vi "Rabi Start.vi"() -> ()   [LabVIEW 2024]
panel:
  in  "Use delay commands?":bool
  in  "T set":string="5E3"
  in  "B Gate Delay":dbl=1.837e-05
  in  "A Gate Delay":dbl=6.308e-06
  in  "stop":bool
  out "At Pass":i32
  in  "MW":dbl=2e-09
  out "Current MW":dbl
  in  "N":dbl=5.0
  out "XY Graph":cluster{"Y":dbl[], "Y":dbl[]}[](graph)
  out "At step":i32
  out "data":dbl[](array[numeric])
  out "A Gate":dbl[][](array[numeric])
  out "B Gate":dbl[][](array[numeric])
  out "DATA":dbl[][](array[numeric])
  in  "Number of steps":i32=500
  in  "Number of individual passes?":i32=10
  in  "Frequency in MHz":string="f2585"
  in  "file path (use dialog)":path=path "C:/Users/Crawford Group/Desktop/DATA (labVIEW Writes)/Rabi/B Gate.txt"
  in  "file path (use dialog) 2":path=path "C:/Users/Crawford Group/Desktop/DATA (labVIEW Writes)/Rabi/A Gate.txt"
  in  "file path (use dialog) 3":path=path "C:/Users/Crawford Group/Desktop/DATA (labVIEW Writes)/Rabi/Averaged.txt"
  # "A gate delay typically at 0.528us\nB gate delay typically at 10.51us"
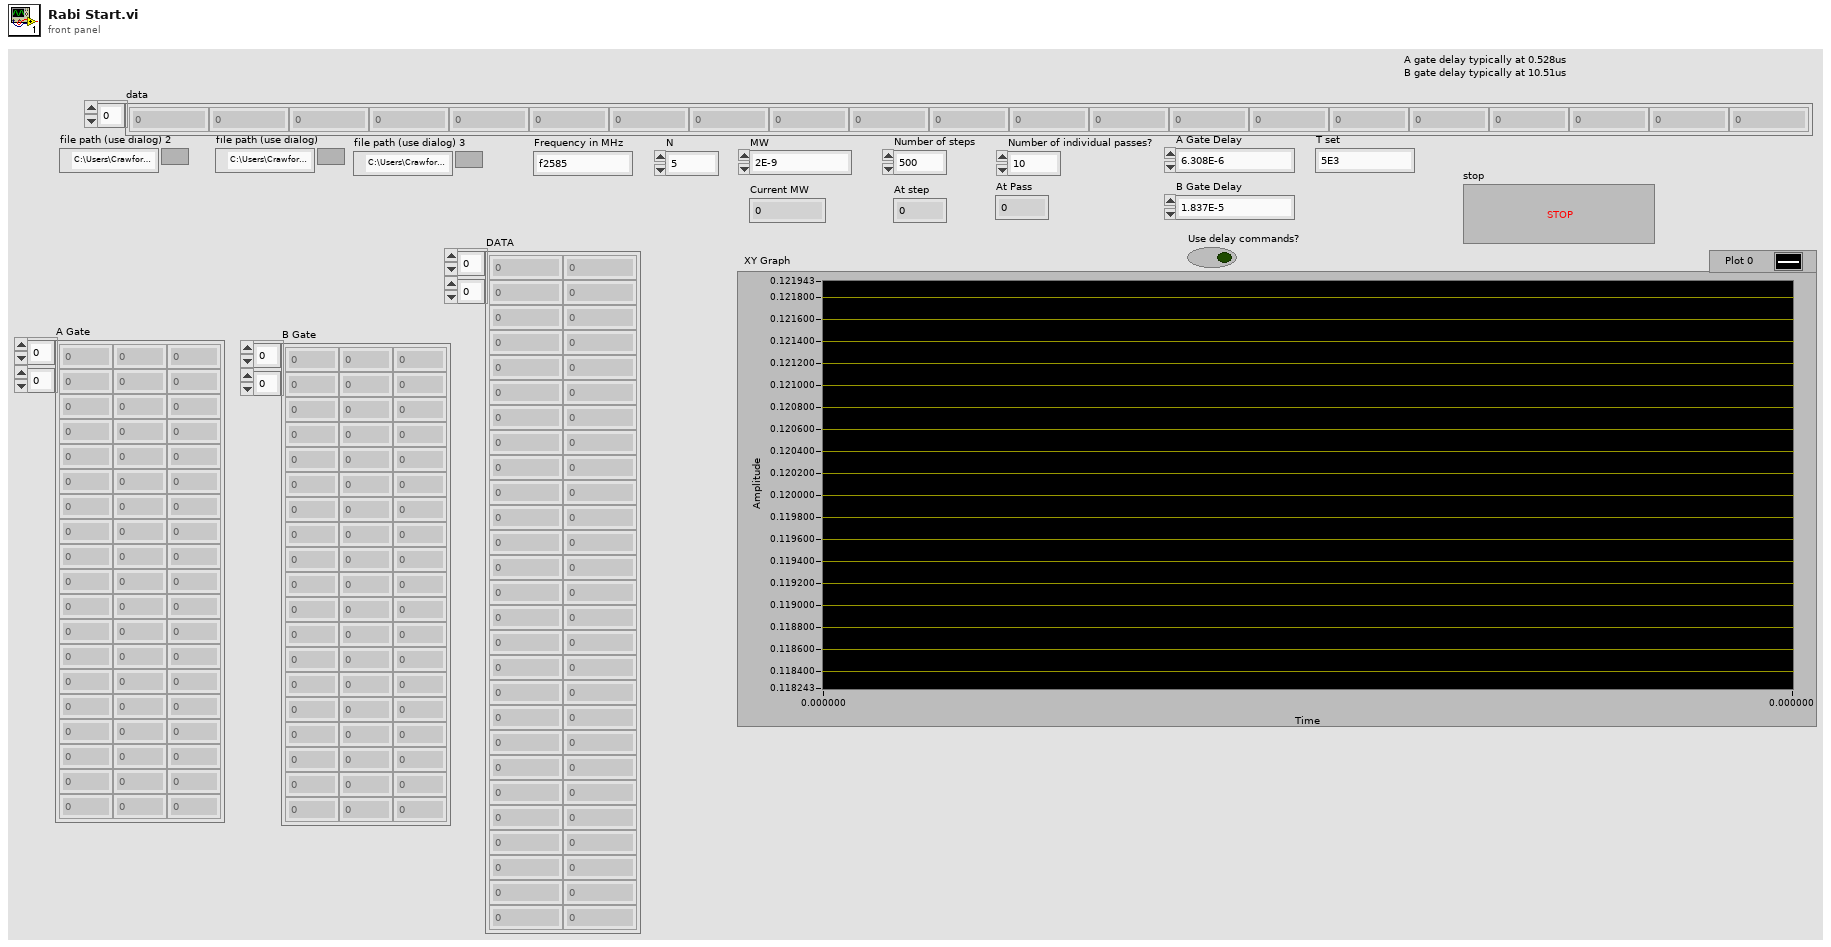
[diagram p1: front panel]
types:
  T1 = enum16{"open", "replace", "create", "open or create", "replace or create", "replace or create with confirmation"}
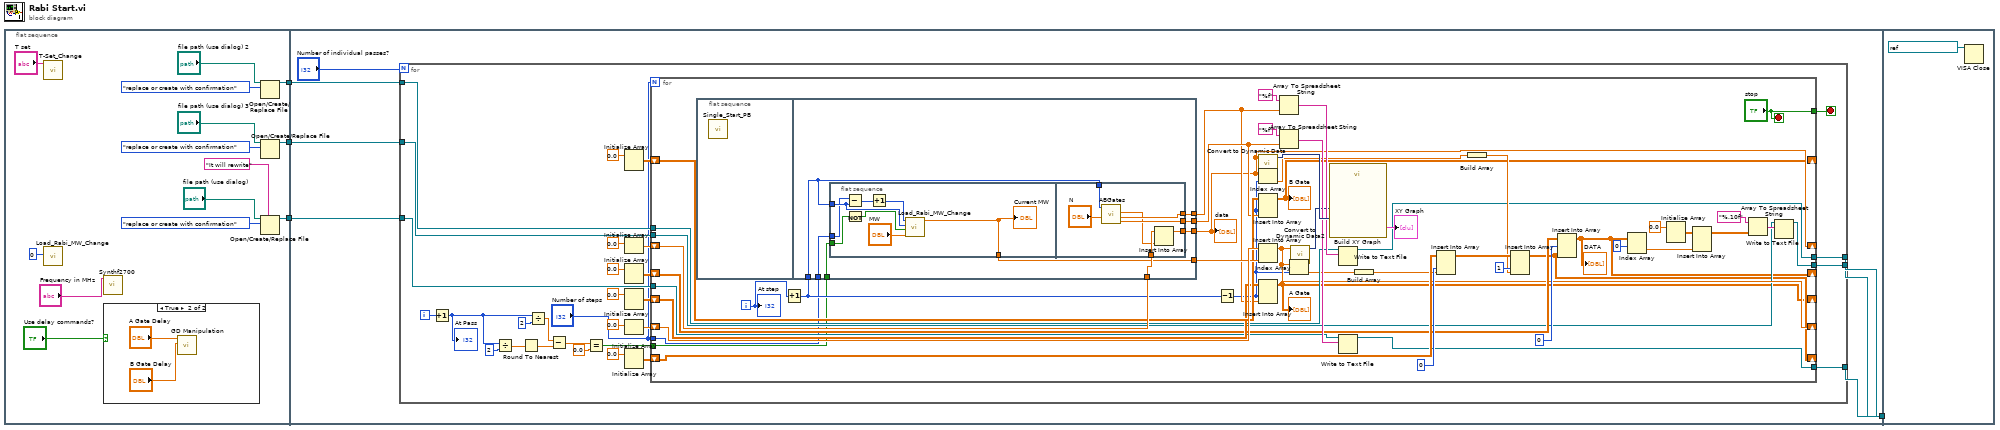
[diagram p0: block diagram]
diagram:
  n1 = flat-sequence {
    tunnel: [w15] -> w6
    tunnel: [w12] -> w5
    tunnel: [w9] -> w4
    tunnel: w6 -> [w29]
    tunnel: w5 -> [w28]
    tunnel: w4 -> [w27]
    tunnel: [w26] -> w3
    tunnel: [w25] -> w2
    tunnel: [w24] -> w1
    tunnel: w3 -> [_]
    tunnel: w2 -> [_]
    tunnel: w1 -> [_]
    frame #0 {
      n2 = call "T-Set_Change.vi"("T set"="T set") -> ()  [unwired: 11 in]
      n3 = call "Load_Rabi_MW_Change.vi"("Numeric"=0) -> ()  [unwired: 9 in, 1 out]
      n4 = call "Synthf2700.vi"("Frequency in MHz"="Frequency in MHz") -> ()  [unwired: 11 in]
      n5 = case shown="True" "Use delay commands?" {
        frame False {
        }
        frame True {
          n6 = call "GD Manipulation.vi"("B Gate delay"="B Gate Delay", "A Gate Delay"="A Gate Delay") -> ()  [unwired: 10 in]
        }
      }
      n7 = Open/Create/Replace File(file path (use dialog)="file path (use dialog) 2", operation (0:open)=T1."replace or create with confirmation") -> (refnum out=w12:refnum<file>)  [unwired: 4 in, 2 out]
      n8 = Open/Create/Replace File(file path (use dialog)="file path (use dialog) 3", operation (0:open)=T1."replace or create with confirmation") -> (refnum out=w9:refnum<file>)  [unwired: 4 in, 2 out]
      n9 = Open/Create/Replace File(file path (use dialog)="file path (use dialog)", prompt="It will rewrite", operation (0:open)=T1."replace or create with confirmation") -> (refnum out=w15:refnum<file>)  [unwired: 3 in, 2 out]
    }
    frame #1 {
      n10 = for {
        N: "Number of individual passes?" -> [_]
        tunnel: w29 -> [w51]
        tunnel: [w44] -> w26
        tunnel: w27 -> [w45]
        tunnel: [w43] -> w25
        tunnel: w28 -> [w50]
        tunnel: [w42] -> w24
        i -> [w38]
        stop <- w30 stop-if-true
        n11 = Increment(x=w38) -> (x+1=w37:i32)
        "At Pass" <- w37
        n12 = Divide(x=w37, y=2) -> (x/y=w34:dbl)
        n13 = Round To Nearest(number=w34) -> (nearest integer value=w33:dbl)
        n14 = Divide(x=w37, y=2) -> (x/y=w39:dbl)
        n15 = Subtract(x=w39, y=w33) -> (x-y=w36:dbl)
        n16 = Equal?(x=w36, y=0.0) -> (x = y?=w32:bool)
        n17 = Initialize Array(0.0) -> (w53:dbl[][])  [unwired: 2 in]
        n18 = Initialize Array(0.0) -> (w59:dbl[])  [unwired: 1 in]
        n19 = Initialize Array(0.0) -> (w46:dbl[][])  [unwired: 2 in]
        n20 = Initialize Array(0.0) -> (w52:dbl[][])  [unwired: 2 in]
        n21 = Initialize Array(0.0) -> (w58:dbl[])  [unwired: 1 in]
        n22 = Initialize Array(0.0) -> (w48:dbl[][])  [unwired: 2 in]
        n23 = for {
          N: "Number of steps" -> [_]
          shift-right: [w81] -> _
          shift-left: w59 -> [w108]
          shift-right: [w86] -> _
          shift-left: w58 -> [w107]
          shift-right: [w61] -> _
          shift-left: w53 -> [w104]
          shift-right: [w60] -> _
          shift-left: w52 -> [w103]
          tunnel: w51 -> [w101]
          tunnel: w50 -> [w97]
          shift-right: [w73] -> _
          shift-left: w48 -> [w91]
          shift-right: [w69] -> _
          shift-left: w46 -> [w90]
          tunnel: w45 -> [w77]
          tunnel: [w68] -> w44
          tunnel: [w67] -> w43
          tunnel: [w66] -> w42
          tunnel: w32 -> [w64]
          tunnel: "Number of steps" -> [w63]
          tunnel: ["stop"] -> w30
          i -> [w65]
          stop <- "stop" stop-if-true
          n24 = flat-sequence {
            tunnel: w87 -> [w114]
            tunnel: w108 -> [w111]
            tunnel: [w110] -> w81
            tunnel: [w109] -> w106
            tunnel: [w112] -> w96
            tunnel: [w113] -> w99
            tunnel: w64 -> [w116]
            tunnel: w63 -> [w115]
            frame #0 {
              n25 = call "Single_Start_PB.vi"() -> ()  [unwired: 12 in]
            }
            frame #1 {
              n26 = flat-sequence {
                tunnel: w114 -> [w124]
                tunnel: w116 -> [w123]
                tunnel: w115 -> [w122]
                tunnel: [w119] -> w109
                tunnel: w114 -> [w130]
                tunnel: [w129] -> w113
                tunnel: [w128] -> w112
                tunnel: w111 -> [w127]
                tunnel: [w125] -> w110
                frame #0 {
                  n27 = Subtract(x=w122, y=w124) -> (x-y=w118:i32)
                  n28 = Not(x=w123) -> (.not. x?=w120:bool)
                  n29 = Increment(x=w118) -> (x+1=w117:i32)
                  n30 = call "Load_Rabi_MW_Change.vi"("Numeric 2"=w117, "Numeric"=w124, 2:w120, "MW Step Size"="MW") -> ("MW"=w119:dbl)  [unwired: 6 in]
                  "Current MW" <- w119
                }
                frame #1 {
                  n31 = call "ABGates.vi"("N"="N", "# of loop"=w130) -> ("B Gate"=w129:dbl[], "A Gate"=w128:dbl[], "average A-B/A+B"=w126:dbl)  [unwired: 7 in]
                  n32 = Insert Into Array(array=w127, new element=w126) -> (w125:dbl[])  [unwired: 1 in]
                }
              }
            }
          }
          n33 = Increment(x=w65) -> (x+1=w87:i32)
          n34 = Decrement(x=w87) -> (x-1=w80:i32)
          n35 = call "Convert to Dynamic Data"("Array"=w81) -> ("Dynamic Data Type"=w105:dynamicdata)  [unwired: 3 in]
          n36 = Index Array(array=w81, index=w80) -> (element=w83:dbl)
          n37 = Insert Into Array(array=w104, index (col)=w80, new element=w99) -> (w61:dbl[][])  [unwired: 1 in]
          "B Gate" <- w61
          n38 = Insert Into Array(array=w107, new element=w106) -> (w86:dbl[])  [unwired: 1 in]
          n39 = Insert Into Array(array=w103, index (col)=w80, new element=w96) -> (w60:dbl[][])  [unwired: 1 in]
          "A Gate" <- w60
          n40 = Array To Spreadsheet String(array=w96, 3:"%f" ("format string")) -> (spreadsheet string=w98:string)  [unwired: 1 in]
          n41 = Array To Spreadsheet String(array=w99, 3:"%f" ("format string")) -> (spreadsheet string=w102:string)  [unwired: 1 in]
          n42 = Index Array(array=w86, index=w80) -> (element=w85:dbl)
          n43 = call "Convert to Dynamic Data2"("Array"=w86) -> ("Dynamic Data Type"=w88:dynamicdata)  [unwired: 3 in]
          n44 = call "Build XY Graph"("Y Input"=w105, "X Input"=w88) -> ("XY Graph"=→"XY Graph":cluster{"X":dbl[], "Y":dbl[]}[])  [unwired: 8 in, 1 out]
          n45 = Write to Text File(file (use dialog)=w97, text=w98) -> (refnum out=w67:refnum<file>)  [unwired: 2 in, 2 out]
          n46 = Write to Text File(file (use dialog)=w101, text=w102) -> (refnum out=w68:refnum<file>)  [unwired: 2 in, 2 out]
          n47 = Build Array(w85) -> (w84:dbl[])
          n48 = Insert Into Array "Insert Into Array"(array=w91, index (col)=0 ("disabled index (col)"), new element=w84) -> (w92:dbl[][])  [unwired: 1 in]
          n49 = Build Array(w83) -> (w82:dbl[])
          n50 = Insert Into Array(array=w92, index (col)=1 ("disabled index (col)"), new element=w82) -> (w73:dbl[][])  [unwired: 1 in]
          n51 = Insert Into Array(array=w90, index (row)=0, new element=w73) -> (w69:dbl[][])  [unwired: 1 in]
          "DATA" <- w69
          n52 = Index Array(array=w69, index (row)=0) -> (element=w71:dbl[])  [unwired: 1 in]
          n53 = Initialize Array(0.0 ("element")) -> (w70:dbl[][])  [unwired: 2 in]
          n54 = Insert Into Array(array=w70, new element=w71) -> (w74:dbl[][])  [unwired: 2 in]
          n55 = Array To Spreadsheet String(array=w74, 3:"%.10f" ("format string")) -> (spreadsheet string=w78:string)  [unwired: 1 in]
          n56 = Write to Text File(file (use dialog)=w77, text=w78) -> (refnum out=w66:refnum<file>)  [unwired: 2 in, 2 out]
          "At step" <- w65
          "data" <- w81
        }
      }
    }
    frame #2 {
      n57 = VISA Close(VISA resource name=refnum<visa-resource-name> "GPIB0::23::INSTR") -> ()  [unwired: 1 in, 1 out]
    }
  }
